vi "BNO055  OPEN.vi"(8 "error in (no error)":errorcluster) -> (0 "error out":errorcluster, 3 "I2C Ref Out":T1)   [LabVIEW 2019]
uses:
  <vilib>/myRIO/Instrument Drivers/Onboard IO/I2C/typedefs/I2C Reference.ctl
  <vilib>/myRIO/Common/Instrument Driver Framework/Utilities/typedefs/myRIO Generic Hardware Reference.ctl
  <vilib>/myRIO/Common/Instrument Driver Framework/Utilities/typedefs/Hardware Version Enum.ctl
  <vilib>/myRIO/Common/Instrument Driver Framework/Utilities/typedefs/myRIO v1.0 Reference.ctl
  <vilib>/myRIO/Common/Instrument Driver Framework/Utilities/typedefs/Generic FPGA Reference.ctl
  <vilib>/myRIO/Common/Instrument Driver Framework/myRIO v1.0/I2C/typedefs/I2C Channels Enum.ctl
  <vilib>/myRIO/Instrument Drivers/Onboard IO/I2C/typedefs/I2C Configuration.ctl
  <vilib>/myRIO/Instrument Drivers/Onboard IO/I2C/typedefs/I2C Transfer Rate.ctl
  <vilib>/myRIO/Instrument Drivers/Onboard IO/I2C/typedefs/I2C User Configuration.ctl
  <vilib>/Utility/error.llb/Error Cluster From Error Code.vi
  <vilib>/myRIO/Common/Instrument Driver Framework/myRIO v1.0/I2C/vis/myRIO v1.0 Configure I2C.vi
  <vilib>/myRIO/Common/Instrument Driver Framework/myRIO v1.0/I2C/vis/myRIO v1.0 Write I2C.vi
  <vilib>/myRIO/Instrument Drivers/Onboard IO/I2C/I2C.lvlib
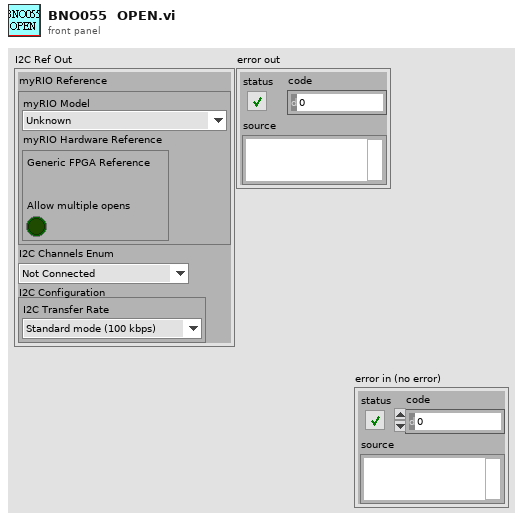
[diagram p1: front panel]
types:
  T1 = typedef "I2C.lvlib/I2C Reference.ctl" = cluster{"myRIO Reference":T2, "I2C Channels Enum":T6, "I2C Configuration":T7}
  T2 = typedef "myRIO Generic Hardware Reference.ctl" = cluster{"myRIO Model":T3, "myRIO Hardware Reference":T4}
  T3 = typedef "Hardware Version Enum.ctl" = enum16{"Unknown", "myRIO-1900", "myRIO-1950", "roboRIO", "NI ELVIS RIO CM", "ELVIS III"}
  T4 = typedef "myRIO v1.0 Reference.ctl" = cluster{"Generic FPGA Reference":T5, "Allow multiple opens":bool}
  T5 = typedef "Generic FPGA Reference.ctl" = refnum<k20>
  T6 = typedef "I2C Channels Enum.ctl" = enum16{"Not Connected", "A/I2C", "B/I2C", "I2C/I2C"}
  T7 = typedef "I2C.lvlib/I2C Configuration.ctl" = cluster{"I2C Transfer Rate":T8}
  T8 = typedef "I2C.lvlib/I2C Transfer Rate.ctl" = enum16{"Standard mode (100 kbps)", "Fast mode (400 kbps)"}
  T9 = typedef "I2C.lvlib/I2C User Configuration.ctl" = cluster{"I2C Transfer Rate":T8}
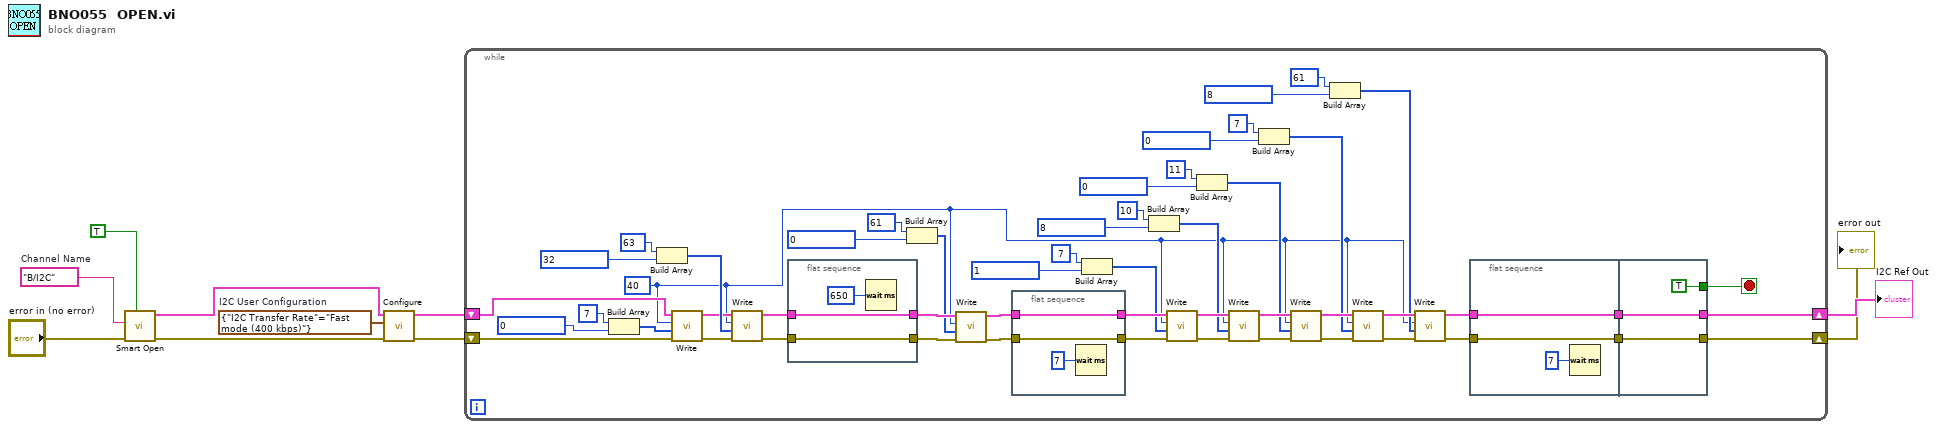
[diagram p0: block diagram]
diagram:
  w4 = T9 {"I2C Transfer Rate"=enum."Fast mode (400 kbps)"}  # I2C User Configuration
  w3 = tag "B/I2C"  # Channel Name
  n1 = call <vilib>:"Smart Open.vi"("Allow multiple opens?"=TRUE, "error in (no error)"="error in (no error)", "Channel Name"=w3) -> ("error out"=w7:errorcluster, "I2C Ref Out"=w6:T1)  [unwired: 7 in]
  n2 = call <vilib>:"Configure.vi"("error in (no error)"=w7, "I2C User Configuration"=w4, "I2C Ref In"=w6) -> ("error out"=w9:errorcluster, "I2C Ref Out"=w8:T1)  [unwired: 7 in]
  n3 = while {
    shift-right: [w18] -> w2
    shift-left: w8 -> [w13]
    shift-right: [w17] -> w1
    shift-left: w9 -> [w14]
    stop <- w19 stop-if-true
    w12 = 40
    n4 = Build Array(7, 0) -> (w11:i32[])
    n5 = Build Array(63, 32) -> (w58:i32[])
    n6 = call <vilib>:"Write.vi"("error in (no error)"=w14, "Bytes to Write"=w11, "Slave Address (7-bit)"=w12, "I2C Ref In"=w13) -> ("error out"=w16:errorcluster, "I2C Ref Out"=w15:T1)  [unwired: 6 in]
    n7 = call <vilib>:"Write.vi"("error in (no error)"=w16, "Bytes to Write"=w58, "Slave Address (7-bit)"=w12, "I2C Ref In"=w15) -> ("error out"=w56:errorcluster, "I2C Ref Out"=w57:T1)  [unwired: 6 in]
    n8 = flat-sequence {
      tunnel: [w73] -> w53
      tunnel: w57 -> [w73]
      tunnel: [w72] -> w52
      tunnel: w56 -> [w72]
      frame #0 {
        n9 = Wait (ms)(milliseconds to wait=u32 650) -> ()  [unwired: 1 out]
      }
    }
    n10 = Build Array(61, 0) -> (w51:i32[])
    n11 = call <vilib>:"Write.vi"("error in (no error)"=w52, "Bytes to Write"=w51, "Slave Address (7-bit)"=w12, "I2C Ref In"=w53) -> ("error out"=w49:errorcluster, "I2C Ref Out"=w50:T1)  [unwired: 6 in]
    n12 = flat-sequence {
      tunnel: [w70] -> w48
      tunnel: w50 -> [w70]
      tunnel: [w69] -> w47
      tunnel: w49 -> [w69]
      frame #0 {
        n13 = Wait (ms)(milliseconds to wait=u32 7) -> ()  [unwired: 1 out]
      }
    }
    n14 = Build Array(7, 1) -> (w44:i32[])
    n15 = Build Array(10, 8) -> (w35:i32[])
    n16 = call <vilib>:"Write.vi"("error in (no error)"=w47, "Bytes to Write"=w44, "Slave Address (7-bit)"=w12, "I2C Ref In"=w48) -> ("error out"=w40:errorcluster, "I2C Ref Out"=w43:T1)  [unwired: 6 in]
    n17 = Build Array(11, 0) -> (w34:i32[])
    n18 = call <vilib>:"Write.vi"("error in (no error)"=w40, "Bytes to Write"=w35, "Slave Address (7-bit)"=w12, "I2C Ref In"=w43) -> ("error out"=w41:errorcluster, "I2C Ref Out"=w42:T1)  [unwired: 6 in]
    n19 = Build Array(7, 0) -> (w29:i32[])
    n20 = call <vilib>:"Write.vi"("error in (no error)"=w41, "Bytes to Write"=w34, "Slave Address (7-bit)"=w12, "I2C Ref In"=w42) -> ("error out"=w32:errorcluster, "I2C Ref Out"=w33:T1)  [unwired: 6 in]
    n21 = Build Array(61, 8) -> (w24:i32[])
    n22 = call <vilib>:"Write.vi"("error in (no error)"=w32, "Bytes to Write"=w29, "Slave Address (7-bit)"=w12, "I2C Ref In"=w33) -> ("error out"=w25:errorcluster, "I2C Ref Out"=w26:T1)  [unwired: 6 in]
    n23 = call <vilib>:"Write.vi"("error in (no error)"=w25, "Bytes to Write"=w24, "Slave Address (7-bit)"=w12, "I2C Ref In"=w26) -> ("error out"=w22:errorcluster, "I2C Ref Out"=w23:T1)  [unwired: 6 in]
    n24 = flat-sequence {
      tunnel: w23 -> [w64]
      tunnel: w22 -> [w63]
      tunnel: [w64] -> w21
      tunnel: [w63] -> w20
      tunnel: [w67] -> w17
      tunnel: [w68] -> w18
      tunnel: w21 -> [w68]
      tunnel: w20 -> [w67]
      tunnel: [TRUE] -> w19
      frame #0 {
        n25 = Wait (ms)(milliseconds to wait=u32 7) -> ()  [unwired: 1 out]
      }
      frame #1 {
      }
    }
  }
  "I2C Ref Out" <- w2
  "error out" <- w1
